vi "Obtain Broadcast Events.vi"(8 "error in":errorcluster, 10 "Create New? (F)":bool) -> (0 "error out":errorcluster, 2 "testCoordinator Broadcast Events":T1)   [LabVIEW 2026, in "testCoordinator.lvlib"]
doc: "This VI Obtains/Creates the Broadcast events that will be used for other modules to register to receive messages from the module that owns this VI.\n\n<b>NOTE</b>: The contents of this VI are automatically generated and modified by the <b>Tools > DQMH Consortium > DQMH</b> utilities. Consider using those utilities instead of making your own modifications to this VI.\n_____\nBased on DQMH Dev Tools: Project Template 7.1.2.1547."
uses:
  testCoordinator.lvlib
  Broadcast Events--cluster.ctl
  Did Init Argument--cluster.ctl
  Status Updated Argument--cluster.ctl
  Error Reported Argument--cluster.ctl
  Do Something Argument--cluster.ctl
  Stop Argument--cluster.ctl
  Get Module Execution Status Argument--cluster.ctl
  Broadcast Available Tests Argument--cluster.ctl
  Refresh Test Procedure Indicator Argument--cluster.ctl
  Refresh Section Indicator Argument--cluster.ctl
  Refresh Instruction Indicator Argument--cluster.ctl
  Broadcast Test Scope Argument--cluster.ctl
  Broadcast Actual Test Procedure Section Argument--cluster.ctl
panel:
  # "NOTE: The contents of this VI are automatically generated and modified by the Tools > DQMH Consortium > DQMH utilities. Consider using those utilities instead of making your own modifications to this VI."
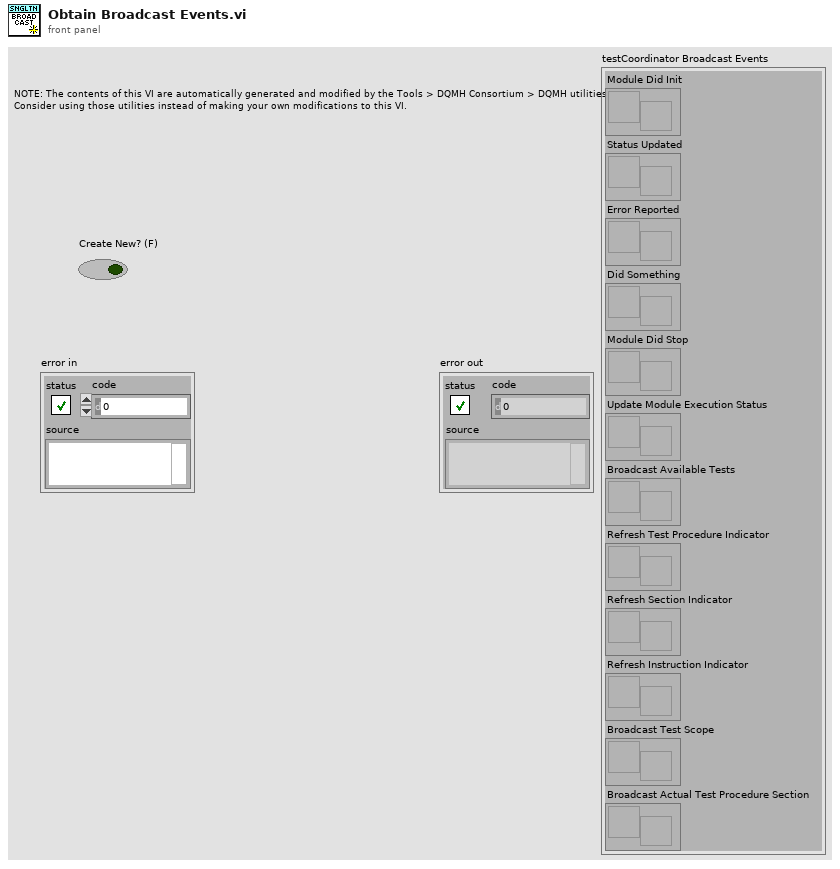
[diagram p1: front panel]
types:
  T1 = typedef "testCoordinator.lvlib/Broadcast Events--cluster.ctl" = cluster{"Module Did Init":refnum<user-event>, "Status Updated":refnum<user-event>, "Error Reported":refnum<user-event>, "Did Something":refnum<user-event>, "Module Did Stop":refnum<user-event>, "Update Module Execution Status":refnum<user-event>, "Broadcast Available Tests":refnum<user-event>, "Refresh Test Procedure Indicator":refnum<user-event>, "Refresh Section Indicator":refnum<user-event>, "Refresh Instruction Indicator":refnum<user-event>, "Broadcast Test Scope":refnum<user-event>, "Broadcast Actual Test Procedure Section":refnum<user-event>}
  T2 = typedef "testCoordinator.lvlib/Broadcast Actual Test Procedure Section Argument--cluster.ctl" = cluster{"Section":string}
  T3 = typedef "testCoordinator.lvlib/Broadcast Test Scope Argument--cluster.ctl" = cluster{"Test Scope":string}
  T4 = typedef "testCoordinator.lvlib/Refresh Instruction Indicator Argument--cluster.ctl" = cluster{"Instruction":string}
  T5 = typedef "testCoordinator.lvlib/Refresh Section Indicator Argument--cluster.ctl" = cluster{"Section":string}
  T6 = typedef "testCoordinator.lvlib/Refresh Test Procedure Indicator Argument--cluster.ctl" = cluster{"Test Procedure":string}
  T7 = typedef "testCoordinator.lvlib/Broadcast Available Tests Argument--cluster.ctl" = cluster{"Available Tests":string[][]}
  T8 = typedef "testCoordinator.lvlib/Get Module Execution Status Argument--cluster.ctl" = cluster{"Running?":bool}
  T9 = typedef "testCoordinator.lvlib/Stop Argument--cluster.ctl" = cluster{"Origin":string, "Exit via Stop Module Req?":bool, "Wait for Module to stop?":bool}
  T10 = typedef "testCoordinator.lvlib/Do Something Argument--cluster.ctl" = cluster{"Do Something Msg":string}
  T11 = typedef "testCoordinator.lvlib/Error Reported Argument--cluster.ctl" = cluster{"Error":errorcluster, "Additional Information":string, "Module Name":string}
  T12 = typedef "testCoordinator.lvlib/Status Updated Argument--cluster.ctl" = cluster{"Status":string}
  T13 = typedef "testCoordinator.lvlib/Did Init Argument--cluster.ctl" = cluster{"Init?":bool, "Info":string}
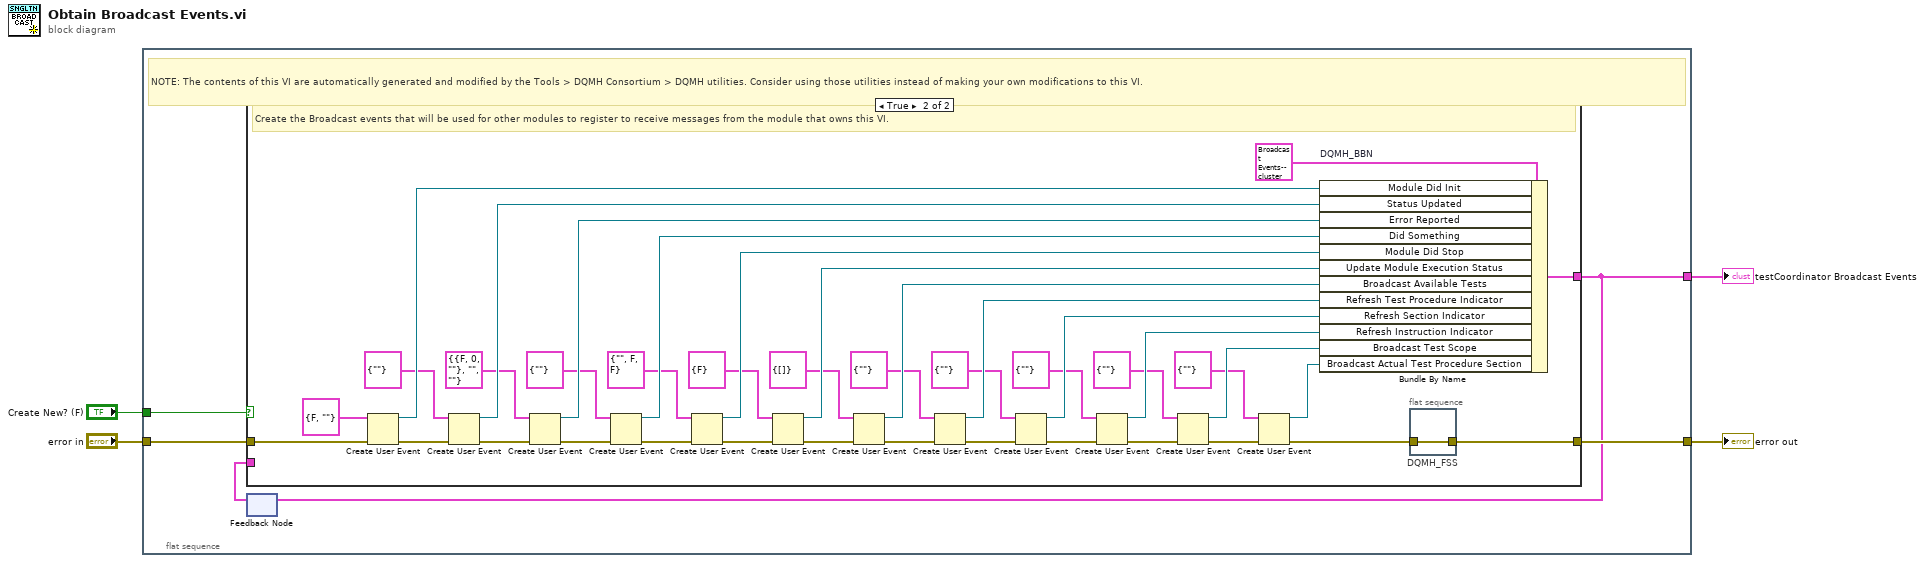
[diagram p0: block diagram]
diagram:
  n1 = flat-sequence {
    tunnel: [w9] -> w4
    tunnel: "error in" -> [w8]
    tunnel: [w6] -> w1
    tunnel: "Create New? (F)" -> [w5]
    frame #0 {
      # "NOTE: The contents of this VI are automatically generated and modified by the Tools > DQMH Consortium > DQMH utilities. Consider using those utilities instead of making your own modifications to this VI."
      n2 = feedback #1() -> (w7:T1)  [unwired: 1 in]
      n3 = case shown="True" w5 {
        tunnel: [w10 w33] -> w9
        tunnel: w8 -> [w10 w51]
        tunnel: [w11 w48] -> w6
        tunnel: w7 -> [w11 _]
        frame False {
          # "Obtain the Broadcast events that were created in a previous call to this VI."
        }
        frame True {
          # "Create the Broadcast events that will be used for other modules to register to receive messages from the module that owns this VI."
          n4 = Create User Event(user event datatype=T13 {"Init?"=FALSE, "Info"=""} ("Did Init Argument"), error in=w51) -> (user event=w49:refnum<user-event>, error out=w46:errorcluster)
          n5 = Create User Event(user event datatype=T12 {"Status"=""} ("Status Updated Argument"), error in=w46) -> (user event=w43:refnum<user-event>, error out=w45:errorcluster)
          n6 = Create User Event(user event datatype=T11 {"Error"={"status"=FALSE, "code"=0, "source"=""}, "Additional Information"="", "Module Name"=""} ("Error Reported Argument"), error in=w45) -> (user event=w40:refnum<user-event>, error out=w42:errorcluster)
          n7 = Create User Event(user event datatype=T10 {"Do Something Msg"=""} ("Did Something"), error in=w42) -> (user event=w38:refnum<user-event>, error out=w37:errorcluster)
          n8 = Create User Event(user event datatype=T9 {"Origin"="", "Exit via Stop Module Req?"=FALSE, "Wait for Module to stop?"=FALSE} ("Stop Argument"), error in=w37) -> (user event=w35:refnum<user-event>, error out=w34:errorcluster)
          n9 = Create User Event(user event datatype=T8 {"Running?"=FALSE} ("Get Module Execution Status Argument"), error in=w34) -> (user event=w31:refnum<user-event>, error out=w32:errorcluster)
          n10 = Create User Event(user event datatype=T7 {"Available Tests"=[]} ("Broadcast Available Tests Argument"), error in=w32) -> (user event=w28:refnum<user-event>, error out=w29:errorcluster)
          n11 = Create User Event(user event datatype=T6 {"Test Procedure"=""} ("Refresh Test Procedure Indicator Argument"), error in=w29) -> (user event=w25:refnum<user-event>, error out=w26:errorcluster)
          n12 = Create User Event(user event datatype=T5 {"Section"=""} ("Refresh Section Indicator Argument"), error in=w26) -> (user event=w22:refnum<user-event>, error out=w23:errorcluster)
          n13 = Create User Event(user event datatype=T4 {"Instruction"=""} ("Refresh Instruction Indicator Argument"), error in=w23) -> (user event=w19:refnum<user-event>, error out=w20:errorcluster)
          n14 = Create User Event(user event datatype=T3 {"Test Scope"=""} ("Broadcast Test Scope Argument"), error in=w20) -> (user event=w16:refnum<user-event>, error out=w17:errorcluster)
          n15 = Create User Event(user event datatype=T2 {"Section"=""} ("Broadcast Actual Test Procedure Section Argument"), error in=w17) -> (user event=w13:refnum<user-event>, error out=w14:errorcluster)
          n16 = Bundle By Name "DQMH_BBN"(cluster=T1 {"Module Did Init"=refnum, "Status Updated"=refnum, "Error Reported"=refnum, "Did Something"=refnum, "Module Did Stop"=refnum, "Update Module Execution Status"=refnum, "Broadcast Available Tests"=refnum, "Refresh Test Procedure Indicator"=refnum, "Refresh Section Indicator"=refnum, "Refresh Instruction Indicator"=refnum, "Broadcast Test Scope"=refnum, "Broadcast Actual Test Procedure Section"=refnum} ("output cluster"), "Module Did Init"=w49, "Status Updated"=w43, "Error Reported"=w40, "Did Something"=w38, "Module Did Stop"=w35, "Update Module Execution Status"=w31, "Broadcast Available Tests"=w28, "Refresh Test Procedure Indicator"=w25, "Refresh Section Indicator"=w22, "Refresh Instruction Indicator"=w19, "Broadcast Test Scope"=w16, "Broadcast Actual Test Procedure Section"=w13) -> (w48:T1)
          n17 = flat-sequence "DQMH_FSS" {
            tunnel: w14 -> [w52]
            tunnel: [w52] -> w33
            frame #0 {
            }
          }
        }
      }
      n18 = feedback-in #1(w6) -> ()
    }
  }
  "error out" <- w4
  "testCoordinator Broadcast Events" <- w1
